vi "To XML.vi"(8 "error in (no error)":errorcluster, 9 "Parent":refnum<k20>, 10 "Document":refnum<k20>, 11 "Line in":refnum<class "Line.lvclass">) -> (0 "error out":errorcluster)   [LabVIEW 2017, in "Cobertura.lvlib" / "Line.lvclass"]
uses:
  Line.lvclass
  Line.lvclass/Line.ctl
  <vilib>/xml/Close Reference(Node).vi
  <resource>/objmgr/DOMUserDefRef.rc
  <vilib>/xml/NI_XML.lvlib
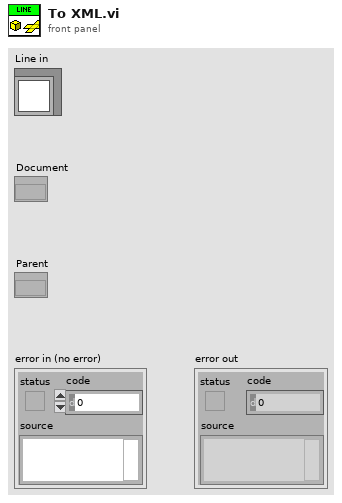
[diagram p1: front panel]
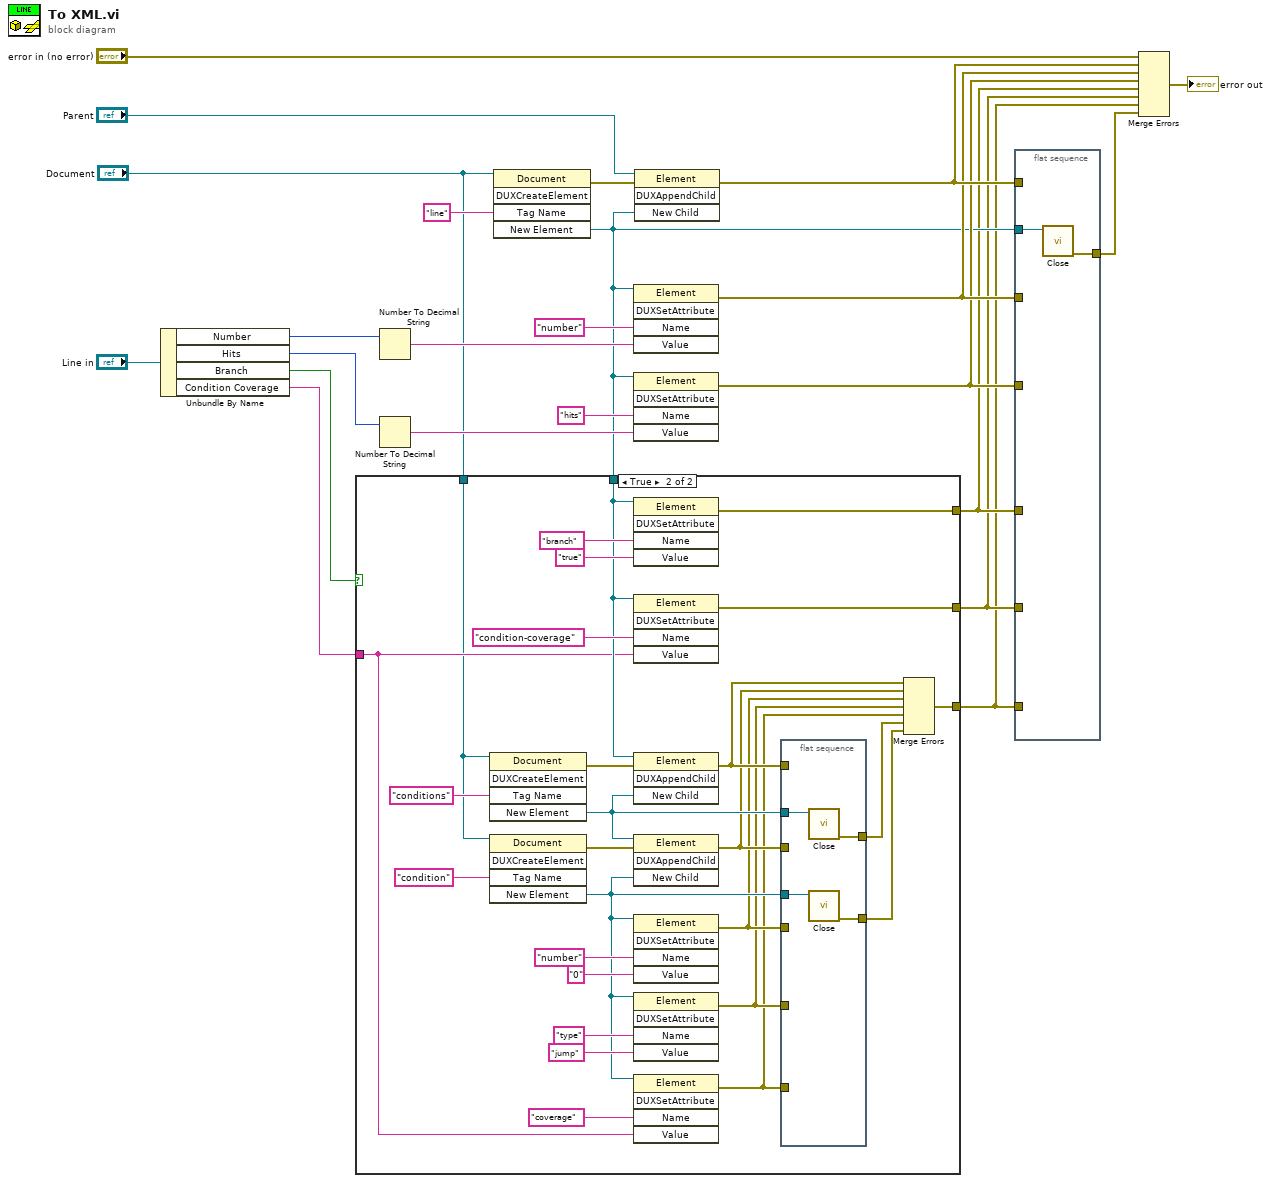
[diagram p0: block diagram]
diagram:
  n1 = Unbundle By Name("Line in") -> ("Number"=w16:u32, "Hits"=w19:u32, "Branch"=w3:bool, "Condition Coverage"=w6:string)
  n2 = Number To Decimal String(number=w16) -> (decimal integer string=w15:string)  [unwired: 1 in]
  n3 = Number To Decimal String(number=w19) -> (decimal integer string=w21:string)  [unwired: 1 in]
  n4 = invoke class="Document" method="DUXCreateElement"(reference="Document", "Tag Name"="line") -> (error out=w14:errorcluster, "New Element"=w7:refnum<k20>)  [unwired: 3 in, 3 out]
  n5 = case shown="True" w3 {
    tunnel: w7 -> [_ w43]
    tunnel: w6 -> [_ w35]
    tunnel: [_ w47] -> w5
    tunnel: [_ w46] -> w4
    tunnel: [_ w25] -> w2
    tunnel: "Document" -> [_ w24]
    frame False {
    }
    frame True {
      n6 = invoke class="Document" method="DUXCreateElement"(reference=w24, "Tag Name"="conditions") -> (error out=w42:errorcluster, "New Element"=w34:refnum<k20>)  [unwired: 3 in, 3 out]
      n7 = invoke class="Document" method="DUXCreateElement"(reference=w24, "Tag Name"="condition") -> (error out=w41:errorcluster, "New Element"=w33:refnum<k20>)  [unwired: 3 in, 3 out]
      n8 = invoke class="Element" method="DUXSetAttribute"(reference=w43, "Name"="branch", "Value"="true" ("Name")) -> (error out=w47:errorcluster)  [unwired: 2 in, 4 out]
      n9 = invoke class="Element" method="DUXSetAttribute"(reference=w43, "Name"="condition-coverage", "Value"=w35) -> (error out=w46:errorcluster)  [unwired: 2 in, 4 out]
      n10 = invoke class="Element" method="DUXAppendChild"(reference=w43, error in=w42, "New Child"=w34) -> (error out=w32:errorcluster)  [unwired: 1 in, 3 out]
      n11 = invoke class="Element" method="DUXAppendChild"(reference=w34, error in=w41, "New Child"=w33) -> (error out=w31:errorcluster)  [unwired: 1 in, 3 out]
      n12 = invoke class="Element" method="DUXSetAttribute"(reference=w33, "Name"="number", "Value"="0") -> (error out=w30:errorcluster)  [unwired: 2 in, 4 out]
      n13 = invoke class="Element" method="DUXSetAttribute"(reference=w33, "Name"="type", "Value"="jump") -> (error out=w29:errorcluster)  [unwired: 2 in, 4 out]
      n14 = invoke class="Element" method="DUXSetAttribute"(reference=w33, "Name"="coverage", "Value"=w35) -> (error out=w28:errorcluster)  [unwired: 2 in, 4 out]
      n15 = flat-sequence {
        tunnel: w34 -> [w54]
        tunnel: [w53] -> w26
        tunnel: w33 -> [w52]
        tunnel: w28 -> [_]
        tunnel: w29 -> [_]
        tunnel: w30 -> [_]
        tunnel: w31 -> [_]
        tunnel: w32 -> [_]
        tunnel: [w51] -> w27
        frame #0 {
          n16 = call-poly <vilib>:"Close.vi"("node"=w54) -> ("error out"=w51:errorcluster)  [unwired: 8 in]
          n17 = call-poly <vilib>:"Close.vi"("node"=w52) -> ("error out"=w53:errorcluster)  [unwired: 8 in]
        }
      }
      n18 = Merge Errors(w32, w31, w30, w29, w28, w27, w26) -> (w25:errorcluster)
    }
  }
  n19 = invoke class="Element" method="DUXSetAttribute"(reference=w7, "Name"="number", "Value"=w15) -> (error out=w9:errorcluster)  [unwired: 2 in, 4 out]
  n20 = invoke class="Element" method="DUXSetAttribute"(reference=w7, "Name"="hits", "Value"=w21) -> (error out=w8:errorcluster)  [unwired: 2 in, 4 out]
  n21 = invoke class="Element" method="DUXAppendChild"(reference="Parent", error in=w14, "New Child"=w7) -> (error out=w10:errorcluster)  [unwired: 1 in, 3 out]
  n22 = flat-sequence {
    tunnel: w7 -> [w56]
    tunnel: [w55] -> w11
    tunnel: w10 -> [_]
    tunnel: w9 -> [_]
    tunnel: w8 -> [_]
    tunnel: w5 -> [_]
    tunnel: w4 -> [_]
    tunnel: w2 -> [_]
    frame #0 {
      n23 = call-poly <vilib>:"Close.vi"("node"=w56) -> ("error out"=w55:errorcluster)  [unwired: 8 in]
    }
  }
  n24 = Merge Errors("error in (no error)", w10, w9, w8, w5, w4, w2, w11) -> (→"error out":errorcluster)
